vi "Configuration Path.vi"(8 "error in (no error)":errorcluster) -> (0 "error out":errorcluster, 2 "section":string, 3 "path":path)   [LabVIEW 2019, in "LV-Data.PGSQL.lvclass"]
uses:
  LV-Data.PGSQL.lvclass
  <vilib>/Utility/sysdir.llb/System Directory Type.ctl
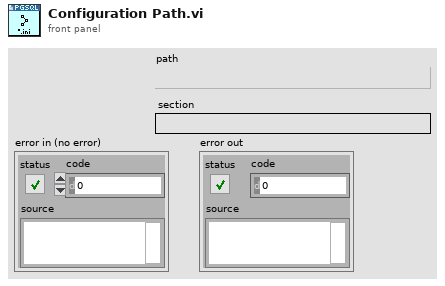
[diagram p1: front panel]
types:
  T1 = typedef "System Directory Type.ctl" = i32
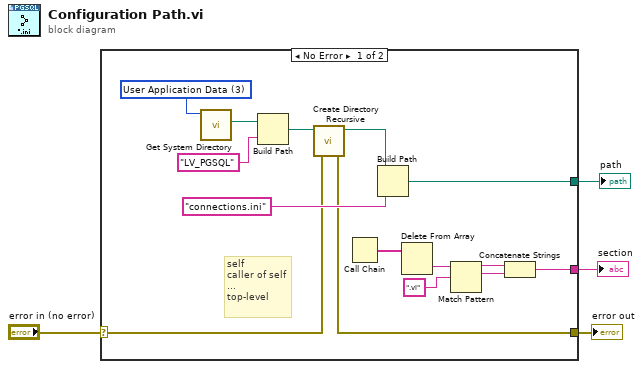
[diagram p0: block diagram]
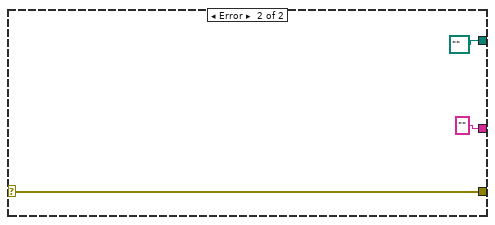
[diagram p2: hidden frame]
diagram:
  n1 = case shown="No Error" "error in (no error)" {
    selector: "error in (no error)" -> [w14 w22]
    tunnel: [w13 w22] -> w4
    tunnel: [w12 path "" ("appended path")] -> w2
    tunnel: [w5 ""] -> w1
    frame No Error {
      w19 = T1 3 items=["User Home"=0, "User Desktop"=1, "User Documents"=2, "User Application Data"=3, "User Preferences"=4, "User Temporary"=5, "Public Documents"=6, "Public Application Data"=7, "Public Preferences"=8, "Public Cache"=13, "System Core Libraries"=9, "System Installed Libraries"=10, "Application Files"=11, "Boot Volume Root"=12] ("system directory type")
      # "self\ncaller of self\n...\ntop-level"
      n2 = call <vilib>:"Get System Directory.vi"("system directory type"=w19) -> ("system directory"=w18:path)  [unwired: 10 in]
      n3 = Build Path(base path=w18, name or relative path="LV_PGSQL") -> (appended path=w11:path)
      n4 = call <vilib>:"Create Directory Recursive.vi"("error in (no error)"=w14, "directory"=w11) -> ("error out"=w13:errorcluster, "directory copy"=w16:path)  [unwired: 3 in, 1 out]
      n5 = Call Chain() -> (call chain=w9:string[])
      n6 = Build Path(base path=w16, name or relative path="connections.ini") -> (appended path=w12:path)
      n7 = Delete From Array(array=w9) -> (deleted portion=w6:string)  [unwired: 2 in, 1 out]
      n8 = Match Pattern(string=w6, regular expression=".vi") -> (before substring=w8:string, match substring=w7:string)  [unwired: 1 in, 2 out]
      n9 = Concatenate Strings(w8, w7) -> (w5:string)
    }
    frame Error {
    }
  }
  "error out" <- w4
  "path" <- w2
  "section" <- w1
